vi "gu_list_folder.vi"(8 "error in":errorcluster, 10 "Encoded Match":T1, 11 "Encoded String":T1) -> (0 "error out":errorcluster, 2 "Encoded Folders":T1[](array[typedef]), 3 "Encoded Files":T1[](array[typedef]))   [LabVIEW 2020, in "G-Unicode.lvlib"]
uses:
  G-Unicode.lvlib
  Types/Encoded UTF-8 String.ctl
  lib/g_unicode_32.dll
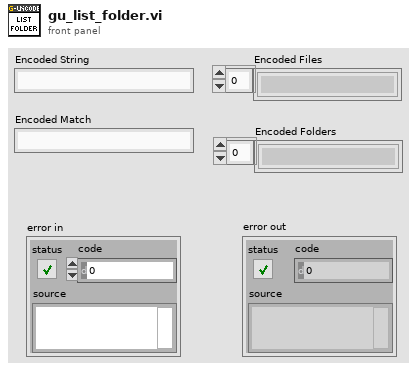
[diagram p1: front panel]
types:
  T1 = typedef "G-Unicode.lvlib/Encoded UTF-8 String.ctl" = string
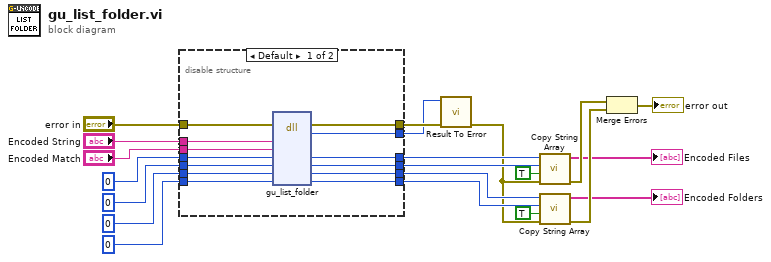
[diagram p0: block diagram]
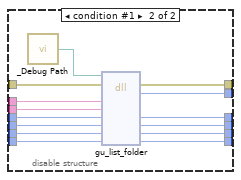
[diagram p2: hidden frame]
diagram:
  n1 = disable-structure shown="Default" {
    disable-tunnel: "Encoded String" -> [w34 w48]
    disable-tunnel: "error in" -> [w33 w47]
    disable-tunnel: [w32 w46] -> w11
    disable-tunnel: i64 0 ("files") -> [w31 w45]
    disable-tunnel: 0 ("num_files") -> [w30 w44]
    disable-tunnel: i64 0 ("folders") -> [w29 w43]
    disable-tunnel: 0 ("num_folders") -> [w28 w42]
    disable-tunnel: [w27 w41] -> w17
    disable-tunnel: [w26 w40] -> w16
    disable-tunnel: [w25 w39] -> w15
    disable-tunnel: [w24 w38] -> w14
    disable-tunnel: "Encoded Match" -> [w23 w36]
    disable-tunnel: [w22 w35] -> w1
    frame condition #0 (active) {
      n2 = dll-call lib="C:/github/dataflowg/g-unicode/src/LabVIEW/G-Unicode/lib/g_unicode_*.*" fn="gu_list_folder"(error in=w33, "path"=w34, "match"=w23, "files"=w31, "num_files"=w30, "folders"=w29, "num_folders"=w28) -> (error out=w32:errorcluster, "result"=w22:i32, "files"=w27:i64, "num_files"=w26:i32, "folders"=w25:i64, "num_folders"=w24:i32)  [unwired: 4 in, 1 out]
    }
    frame condition #1 {
      n3 = call "_Debug Path.vi"() -> ("Debug Path"=w37:path)
      n4 = dll-call lib="?" fn="gu_list_folder"(path in=w37, error in=w47, "path"=w48, "match"=w36, "files"=w45, "num_files"=w44, "folders"=w43, "num_folders"=w42) -> (error out=w46:errorcluster, "result"=w35:i32, "files"=w41:i64, "num_files"=w40:i32, "folders"=w39:i64, "num_folders"=w38:i32)  [unwired: 3 in, 1 out]
    }
  }
  n5 = call "Result To Error.vi"("error in (no error)"=w11, "Result Code"=w1) -> ("error out"=w2:errorcluster)  [unwired: 9 in]
  n6 = call "Copy String Array.vi"("error in"=w2, "free (F)"=TRUE, "size"=w16, "pointer"=w17) -> ("error out"=w10:errorcluster, "Strings"=→"Encoded Files":string[])  [unwired: 6 in]
  n7 = call "Copy String Array.vi"("error in"=w2, "free (F)"=TRUE, "size"=w14, "pointer"=w15) -> ("error out"=w9:errorcluster, "Strings"=→"Encoded Folders":string[])  [unwired: 6 in]
  n8 = Merge Errors(w10, w9) -> (→"error out":errorcluster)
